vi "Observe.vi"(6 "Labels":map{string, string}(c390), 8 "error in (no error)":errorcluster, 10 "New Value":dbl, 11 "Histogram Ref":refnum<data-value>) -> (0 "error out":errorcluster, 3 "Histogram Ref out":refnum<data-value>)   [LabVIEW 2020, in "Metrics.lvlib" / "Histogram.lvclass"]
doc: "Sets the metric value. The histogram metric then updates the number of times bucket values were exceeded by this new value. That is, for each bucket value that are less than the newly observed value, we increment the counter for this treshold value."
uses:
  Histogram.lvclass
  C:/Github-locals/PromVIEW/src/metrics/metric/Metric.lvclass
  Histogram.lvclass/Histogram.ctl
  <vilib>/Utility/miscctls.llb/LVMapReplaceAction.ctl
  sample/Edit Action.ctl
  metric/Metric.lvclass/Metric.ctl
  metric/Write Samples 2.vi
  metric/Metric.lvclass
  sample/Sample.lvclass
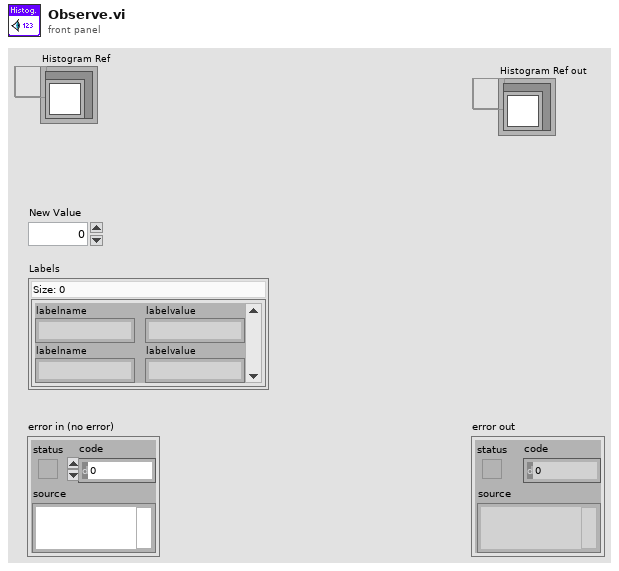
[diagram p1: front panel]
types:
  T1 = typedef "LVMapReplaceAction.ctl" = enum32{"Modify Entry only if found", "Add or Modify Entry", "Delete Entry"}
  T2 = typedef "Metrics.lvlib/Sample.lvclass/Edit Action.ctl" = enum16{"Set", "Increment"}
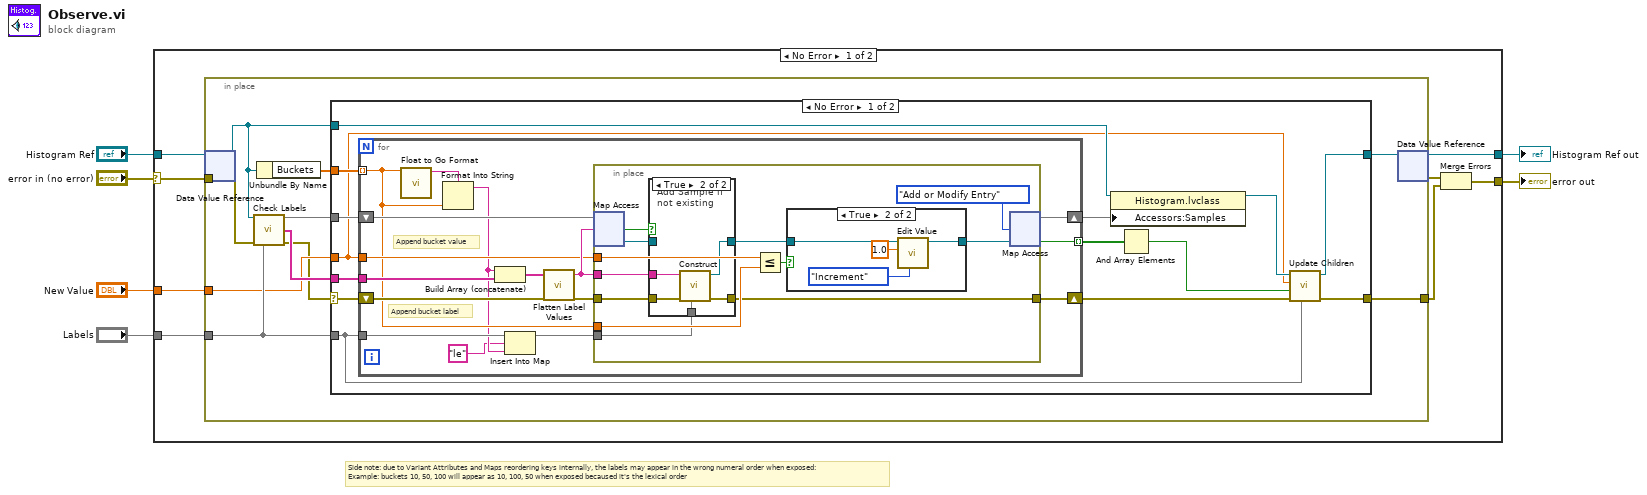
[diagram p0: block diagram]
diagram:
  # "Side note: due to Variant Attributes and Maps reordering keys internally, the labels may appear in the wrong numeral order when exposed:\nExample: buckets 10, 50, 100 will appear as 10, 100, 50 when exposed becaused it's the lexical order"
  n1 = case shown="No Error" "error in (no error)" {
    selector: "error in (no error)" -> [w11 w81]
    tunnel: [w7 w81] -> w5
    tunnel: [w10 w80] -> w2
    tunnel: "Histogram Ref" -> [w14 w80]
    tunnel: "New Value" -> [w12 _]
    tunnel: "Labels" -> [w13 _]
    frame No Error {
      n2 = in-place {
        in-place-border: w13 -> [w22]
        in-place-border: w12 -> [w21]
        in-place-border: w11 -> [w16]
        in-place-border: [w17] -> w8
        n3 = in-place-dvr #1(w14) -> (w19:refnum<class "Histogram.lvclass">)  [unwired: 1 out]
        n4 = call-dynamic "Check Labels.vi"("Histogram in"=w19, "error in (no error)"=w16, "Labels"=w22) -> ("Samples"=w23:map{string, refnum<class "Sample.lvclass">}, "Label Values"=w24:string[], "error out"=w15:errorcluster)  [unwired: 9 in, 1 out]
        n5 = Unbundle By Name(w19) -> ("Buckets"=w18:dbl[])
        n6 = case shown="No Error" w15 {
          selector: w15 -> [w36 w78]
          tunnel: w24 -> [w38 _]
          tunnel: w23 -> [w37 _]
          tunnel: w21 -> [w28 _]
          tunnel: w22 -> [w25 _]
          tunnel: [w26 w78] -> w17
          tunnel: w19 -> [w34 w79]
          tunnel: [w31 w79] -> w20
          tunnel: w18 -> [w33 _]
          frame No Error {
            n7 = for {
              tunnel: w38 -> [w47]
              tunnel: w28 -> [w51]
              tunnel: w25 -> [w42]
              shift-right: [w44] -> w27
              shift-left: w36 -> [w50]
              shift-right: [w49] -> w35
              shift-left: w37 -> [w53]
              tunnel: w33 -> [w45] mode=indexing
              tunnel: [w43] -> w30 mode=indexing
              # "Append bucket label"
              # "Append bucket value"
              n8 = call "Float to Go Format.vi"("Float Value"=w45) -> ("Go Format"=w48:string)  [unwired: 10 in]
              n9 = Format Into String(format string=w48, w45) -> (resulting string=w40:string)  [unwired: 2 in, 1 out]
              n10 = Build Array (concatenate)(w40, w47) -> (w46:string[])
              n11 = Insert Into Map(map in=w42, key="le", value=w40) -> (map out=w41:map{string, string})  [unwired: 2 out]
              n12 = call "Flatten Label Values.vi"("Label Values"=w46) -> ("Flattened labelvalues"=w52:string)  [unwired: 4 in]
              n13 = in-place {
                in-place-border: w52 -> [w57]
                in-place-border: w51 -> [w63]
                in-place-border: w41 -> [w56]
                in-place-border: w50 -> [w55]
                in-place-border: w45 -> [w62]
                in-place-border: [w54] -> w44
                n14 = in-place-map #2(w53, w52) -> (w58:refnum<class "Sample.lvclass">, w60:bool)  [unwired: 1 in]
                n15 = case shown="True" w60 {
                  tunnel: [w72 w77] -> w59
                  tunnel: w58 -> [w72 _]
                  tunnel: w57 -> [_ w76]
                  tunnel: w56 -> [_ w75]
                  tunnel: w55 -> [w71 w74]
                  tunnel: [w71 w73] -> w54
                  frame False {
                  }
                  frame True {
                    # "Add Sample if not existing"
                    n16 = call "Construct.vi"("Labels"=w75, "error in (no error)"=w74, "Name"=w76) -> ("error out"=w73:errorcluster, "Sample out"=w77:refnum<class "Sample.lvclass">)  [unwired: 7 in]
                  }
                }
                n17 = Less Or Equal?(x=w63, y=w62) -> (x <= y?=w61:bool)
                n18 = case shown="True" w61 {
                  tunnel: [w66 w67] -> w64
                  tunnel: w59 -> [w66 w70]
                  frame False {
                  }
                  frame True {
                    n19 = call "Edit Value.vi"("Action"=Edit_Action."Increment", "New Val"=1.0, "Sample in"=w70) -> ("Sample out"=w67:refnum<class "Sample.lvclass">)  [unwired: 7 in, 1 out]
                  }
                }
                n20 = in-place-map #2(w64, LVMapReplaceAction."Add or Modify Entry" ("action")) -> (w49:map{string, refnum<class "Sample.lvclass">}, w43:bool)  [unwired: 1 out]
              }
            }
            n21 = property class="Histogram.lvclass"(reference=w34, "Accessors:Samples"=w35) -> (reference out=w32:refnum<class "Histogram.lvclass">)  [unwired: 1 in, 1 out]
            n22 = And Array Elements(Boolean array=w30) -> (logical AND=w29:bool)
            n23 = call "Update Children.vi"("Labels"=w25, "error in (no error)"=w27, "Created?"=w29, "New Value"=w28, "Histogram in"=w32) -> ("error out"=w26:errorcluster, "Histogram out"=w31:refnum<class "Histogram.lvclass">)  [unwired: 5 in]
          }
          frame Error {
          }
        }
        n24 = in-place-dvr #1(w20) -> (w10:refnum<data-value>, w9:errorcluster)
      }
      n25 = Merge Errors(w9, w8) -> (w7:errorcluster)
    }
    frame Error {
    }
  }
  "error out" <- w5
  "Histogram Ref out" <- w2
